vi "Update Format Labels.vi"(7 "Format Cluster":T1, 8 "error in (no error)":errorcluster, 11 "State In":T2={"Measure ?"=[], "Direction"=[], "Loop ?"={"Start"=0, "Finish"=2}, "Storage Location"=[], "Show Current Location"=FALSE, "Current Location"=0, "Show y=0"=FALSE, "Program"=[], "Index"=0, "Average During Loop ?"=FALSE, "# of Loops"=1, "Loop Control"={0, 2}, "Units"="", "Digits"=0, "Significant Figures (F) or DP (T)"=FALSE, "Rate Mode"=FALSE, "Current Y value"=0.0, "Initial Value"=0.0, "Rate Unit"=""} caption="State" {"# of Loops" min=1 step=1; "Index" min=0 step=1; "Program"."Step" min=0.001 max=80.0 step=0.001 format="%.2f"; "Program"."Target" format="%.2f"}) -> (0 "error out":errorcluster, 3 "State Out":T2={"Measure ?"=[], "Direction"=[], "Loop ?"={"Start"=0, "Finish"=2}, "Storage Location"=[], "Show Current Location"=FALSE, "Current Location"=0, "Show y=0"=FALSE, "Program"=[], "Index"=0, "Average During Loop ?"=FALSE, "# of Loops"=1, "Loop Control"={0, 2}, "Units"="", "Digits"=0, "Significant Figures (F) or DP (T)"=FALSE, "Rate Mode"=FALSE, "Current Y value"=0.0, "Initial Value"=0.0, "Rate Unit"=""} caption="State" {"# of Loops" min=1 step=1; "Index" min=0 step=1; "Program"."Step" min=0.001 max=80.0 step=0.001 format="%.2f"; "Program"."Target" format="%.2f"})   [LabVIEW 2012, in "Multi Segment Waveform.xctl"]
doc: "Updates the labels and format strings of the facade based on the current state of the XControl."
uses:
  Multi Segment Waveform.xctl
  State.ctl
  Type Defs/Formatting Refs.ctl
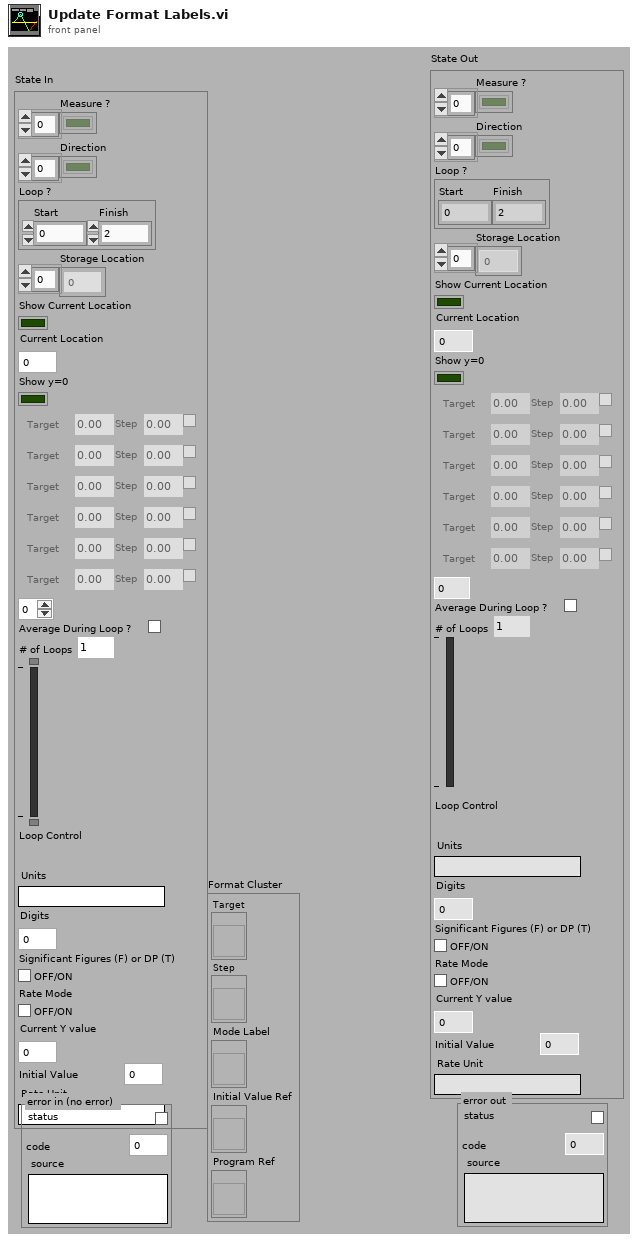
[diagram p1: front panel]
types:
  T1 = typedef "Multi Segment Waveform.xctl/Formatting Refs.ctl" = cluster{"Target":refnum<vi>, "Step":refnum<vi>, "Mode Label":refnum<vi>, "Initial Value Ref":refnum<vi>, "Program Ref":refnum<vi>}
  T2 = typedef "Multi Segment Waveform.xctl/State.ctl" = cluster{"Measure ?":bool[], "Direction":bool[], "Loop ?":cluster{"Start":i32, "Finish":i32}, "Storage Location":i32[], "Show Current Location":bool, "Current Location":i32, "Show y=0":bool, "Program":cluster{"Target":dbl, "Step":dbl, "Measure ?":bool}[], "Index":i32, "Average During Loop ?":bool, "# of Loops":u32, "Loop Control":cluster{i32, i32}, "Units":string, "Digits":i32, "Significant Figures (F) or DP (T)":bool, "Rate Mode":bool, "Current Y value":dbl, "Initial Value":dbl, "Rate Unit":string}
  T3 = cluster{"Target":dbl, "Step":dbl, "Measure ?":bool}[]
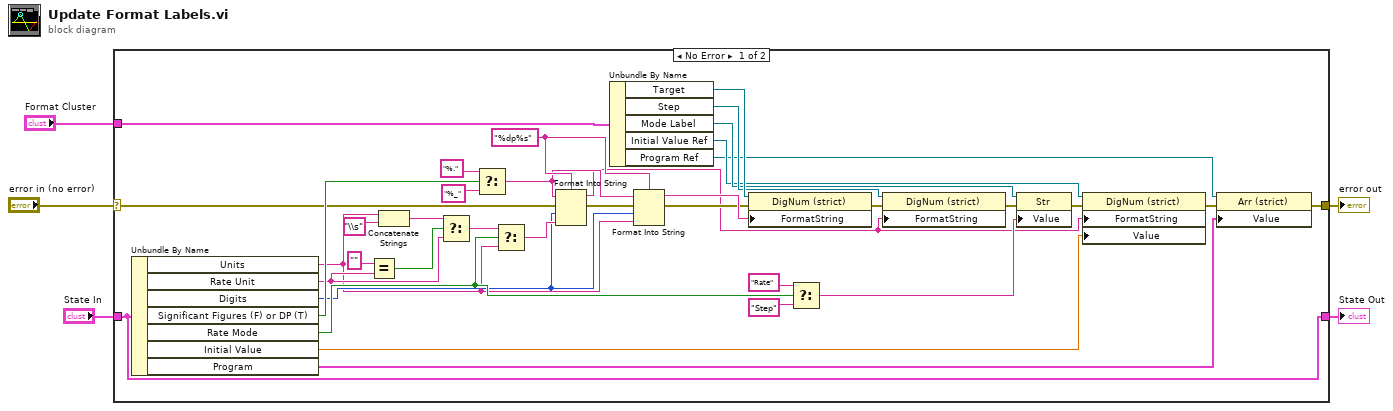
[diagram p0: block diagram]
diagram:
  n1 = case shown="No Error" "error in (no error)" {
    selector: "error in (no error)" -> [w39 w44]
    tunnel: [w13 w44] -> w4
    tunnel: "State In" -> [w34 w43]
    tunnel: "Format Cluster" -> [w38 _]
    tunnel: [w34 w43] -> w1
    frame No Error {
      w24 = "%dp%s" ("format string")
      n2 = Unbundle By Name(w34) -> ("Units"=w7:string, "Rate Unit"=w8:string, "Digits"=w25:i32, "Significant Figures (F) or DP (T)"=w42:bool, "Rate Mode"=w32:bool, "Initial Value"=w17:dbl, "Program"=w14:T3)
      n3 = Equal?(x="", y=w8) -> (x = y?=w11:bool)
      n4 = Concatenate Strings(w7, "\\s" ("string")) -> (w9:string)
      n5 = Select(t=w9, s=w11, f=w8) -> (s? t:f=w6:string)
      n6 = Select(t="%.", s=w42, f="%_") -> (s? t:f=w21:string)
      n7 = Select(t=w6, s=w32, f=w7) -> (s? t:f=w33:string)
      n8 = Format Into String(format string=w24, initial string=w21, error in=w39, w25, w33) -> (resulting string=w18:string, error out=w26:errorcluster)
      n9 = Unbundle By Name(w38) -> ("Target"=w37:refnum<vi>, "Step"=w35:refnum<vi>, "Mode Label"=w28:refnum<vi>, "Initial Value Ref"=w19:refnum<vi>, "Program Ref"=w15:refnum<vi>)
      n10 = Format Into String(format string=w24, initial string=w21, error in=w26, w25, w7) -> (resulting string=w23:string, error out=w22:errorcluster)
      n11 = property class="DigNum (strict)"(reference=w37, error in=w22, "FormatString"=w23) -> (error out=w36:errorcluster)  [unwired: 1 out]
      n12 = Select(t="Rate", s=w32, f="Step") -> (s? t:f=w27:string)
      n13 = property class="DigNum (strict)"(reference=w35, error in=w36, "FormatString"=w18) -> (error out=w29:errorcluster)  [unwired: 1 out]
      n14 = property class="Str"(reference=w28, error in=w29, "Value"=w27) -> (error out=w20:errorcluster)  [unwired: 1 out]
      n15 = property class="DigNum (strict)"(reference=w19, error in=w20, "FormatString"=w18, "Value"=w17) -> (error out=w16:errorcluster)  [unwired: 1 out]
      n16 = property class="Arr (strict)"(reference=w15, error in=w16, "Value"=w14) -> (error out=w13:errorcluster)  [unwired: 1 out]
    }
    frame Error {
    }
  }
  "State Out" <- w1
  "error out" <- w4
